vi "Libray.Connect_to_SNDB.vi"(0 "Log In Data":cluster{"Username":string, "Password":string}, 1 "Command":T2=enum."Initialize HTTPS", 2 "Curl":string="https://srv-sndb.iesy.com", 5 "Serial Number":string, 7 "Update step":T1, 11 "Fehler (Eingang, kein Fehler)":errorcluster, 12 "Input String":string, 13 "Type of the uploaded file":enum16{"txt", "pdf", "image/jpeg"}(ring)) -> (4 "Successful?":bool, 6 "body":string, 8 "headers":string, 15 "error out":errorcluster)   [LabVIEW 2026, in "Connect_to_SNDB_library.lvlib"]
uses:
  Connect_to_SNDB_library.lvlib
  Libray.Connect_to_SNDB_Command.ctl
  <vilib>/httpClient/ClientHandle.ctl
  <vilib>/JDP Science/JSONtext/Next JSON Value.vi
  <vilib>/JDP Science/JSONtext/String Subset.vi
  <vilib>/JDP Science/JSONtext/support/Strip Quotes and Unescape.vi
  <vilib>/JDP Science/JSONtext/Parsing/Advance past next JSON Value (inlined COPY).vi
  <vilib>/JDP Science/JSONtext/support/Unescape JSON string.vi
  <vilib>/JDP Science/JSONtext/Parsing/Advance past whitespace.vi
  <vilib>/JDP Science/JSONtext/Parsing/Advance past String.vi
  <vilib>/JDP Science/JSONtext/Parsing/Advance past Number.vi
  <vilib>/JDP Science/JSONtext/Parsing/Advance past Line Ending.vi
  <vilib>/JDP Science/JSONtext/support/Format JSON Object.vi
  <vilib>/httpClient/POSTBuffer.vi
  <vilib>/JDP Science/JSONtext/Parsing/Parse Full Path or Item Name.vi
  <vilib>/JDP Science/JSONtext/Parsing/Advance past Array.vi
  <vilib>/JDP Science/JSONtext/Parsing/Advance past Object.vi
  <vilib>/JDP Science/JSONtext/support/Error Cluster From Code.vi
  <vilib>/JDP Science/JSONtext/Offset/Find Item Locations by Path.vi
  <vilib>/httpClient/LabVIEWHTTPClient.lvlib
  <vilib>/JDP Science/JSONtext/JSONtext.lvlib
panel:
  out "MAC_Status_Array(with\"\")":string[](array[string])
  out "MAC_Array(with\"\")":string[](array[string])
  out "-H":string
  # "SNDB Libray"
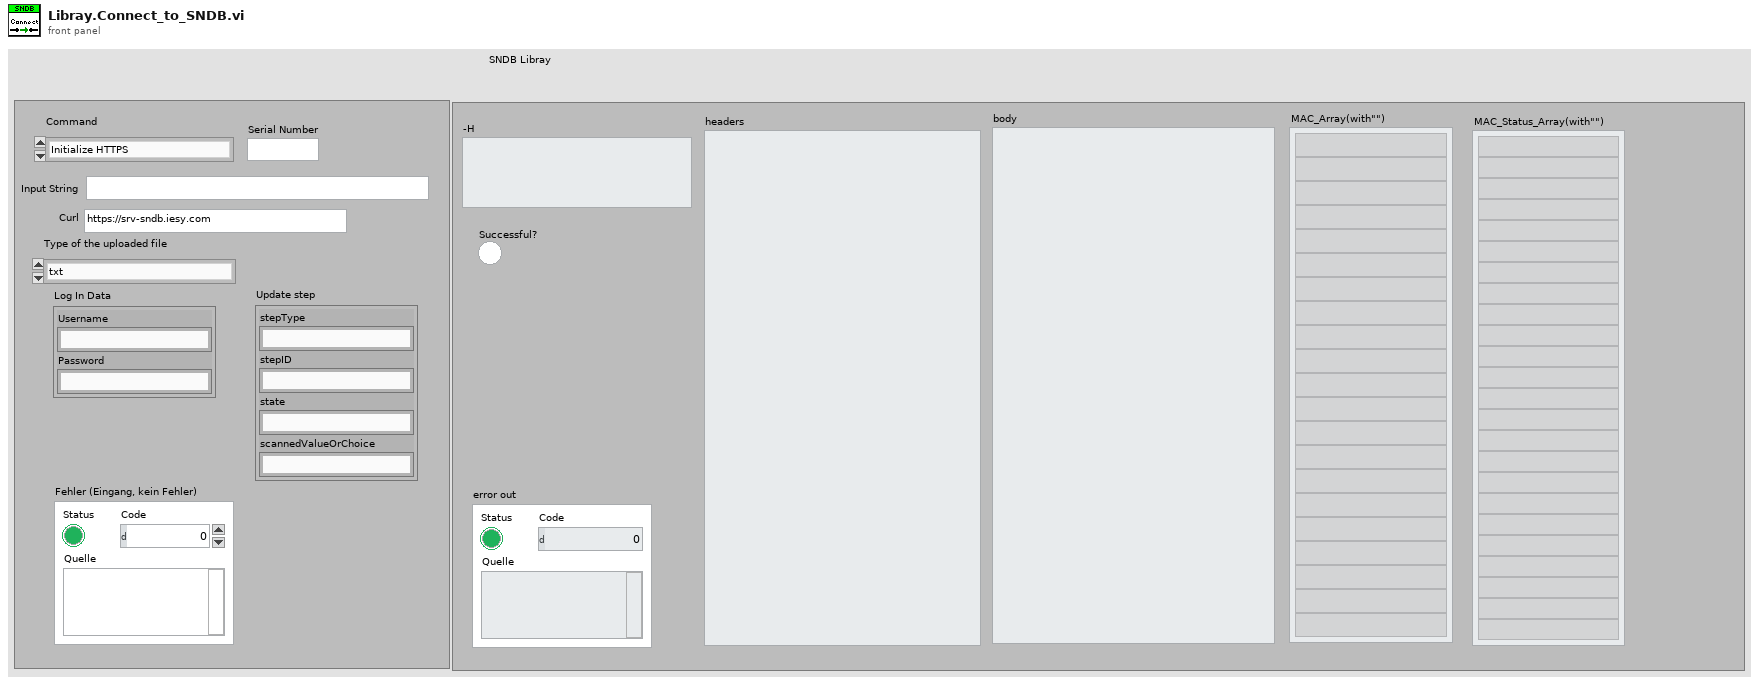
[diagram p1: front panel]
types:
  T1 = cluster{"stepType":string, "stepID":string, "state":string, "scannedValueOrChoice":string}
  T2 = typedef "Connect_to_SNDB_library.lvlib/Libray.Connect_to_SNDB_Command.ctl" = enum16{"No command", "Initialize HTTPS", "Authentication: Creat a token", "Authentication: Get all tokens", "Authentication: Revoke the token", "Label: Creat a label configuration", "Label: Get all configured labels", "Label: Update the label configuration", "Label: Delete the label configuration", "Label: Creat a colour ribbon", "Label: Update the colour ribbon", "Label: Get all colour ribbons", "Label: Delete the colour ribbon", "Label: Creat a label tape", "Label: Update the label tape", "Label: Get all label tapes", "Label: Delete the label tape", "Label: Get all label parameters", "Product: Get all product informations", "Product: Get all reading steps", "Seriennummer: Update the info text", "Seriennummer: Set all step states open", "Seriennummer: Update step states", "Seriennummer: Get data and steps", "Seriennummer: Get all label configurations", "Seriennummer: Create a text report(Prüfbericht)", "Seriennummer: Get the text report(Prüfbericht)", "Seriennummer: Delete the text report(Prüfbericht)", "Seriennummer: Upload a document(txt file)", "Seriennummer: Get the document", "Seriennummer: Get the document thumbnail", "Seriennummer: Delete the document", "Seriennummer: Bulk lookup", "Vorgang: Update the description text", "Vorgang: Migrate serial numbers to a Vorgang", "Vorgang: Migrate serial numbers to a product revision", "Vorgang: Update step states", "Vorgang: Create test reports(Prüfprotokoll)", "Vorgang: Get basic data", "Vorgang: Get serial number data and steps", "Vorgang: Get all serial numbers", "Vorgang: Generate a CSV file", "Vorgang: Generate an XLSX file", "Vorgang: Get a CSV file(Fertigmeldung report)", "Fertigmeldung: Create a Fertigmeldung", "Fertigmeldung: Revert the Fertigmeldung", "User: Get all users", "User: Update an user", "User: Get a single user", "User: Get all user roles", "User: Update a user role", "User: Get a single user role", "User: Get all permissions", "Search: Get Vorgang/Produkt combinations", "Search: Get Vorgang/Produkt/SN combinations", "Search: Get Seriennummern by Vorgang and Produkt", "Search: Lookup Vorgang", "MAC addresses: Get all reserved MAC addresses", "MAC addresses: Get the most recently reserved MAC addresses", "MAC addresses: Get data for a MAC address", "MAC addresses: Reserve a number of MAC addresses for a Seriennummer", "MAC addresses: Make a reserved MAC address as flashed", "Deinitialize HTTPs"}
  T3 = typedef "LabVIEWHTTPClient.lvlib/ClientHandle.ctl" = refnum<k1>
  T4 = cluster{"Name":string, "Value":string, "File":path, "Filename":string, "MIME type":string}
  T5 = cluster{"Name":string, "Value":string, "File":path, "Filename":string, "MIME type":string}[]
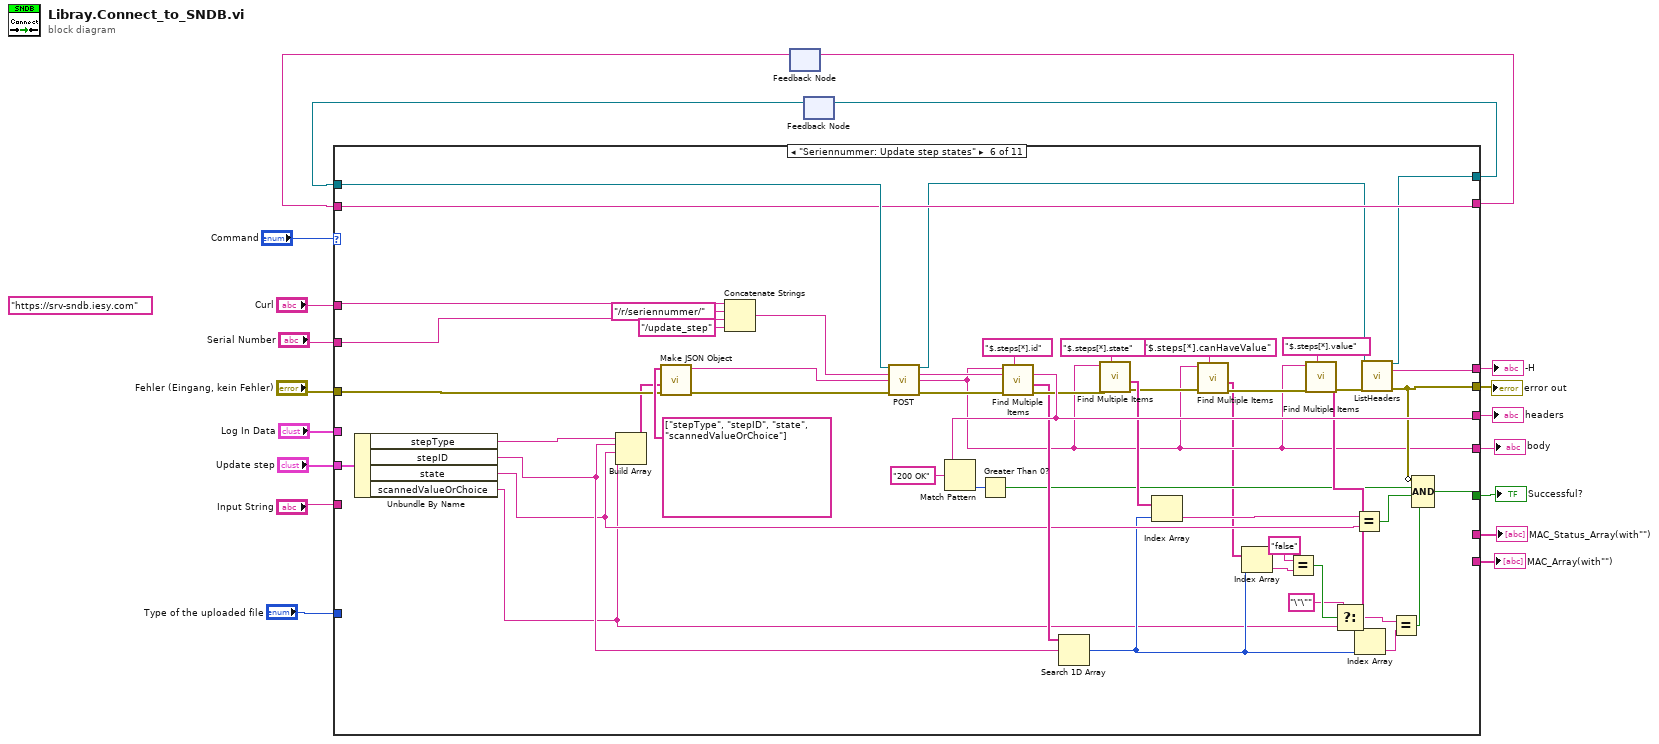
[diagram p0: block diagram]
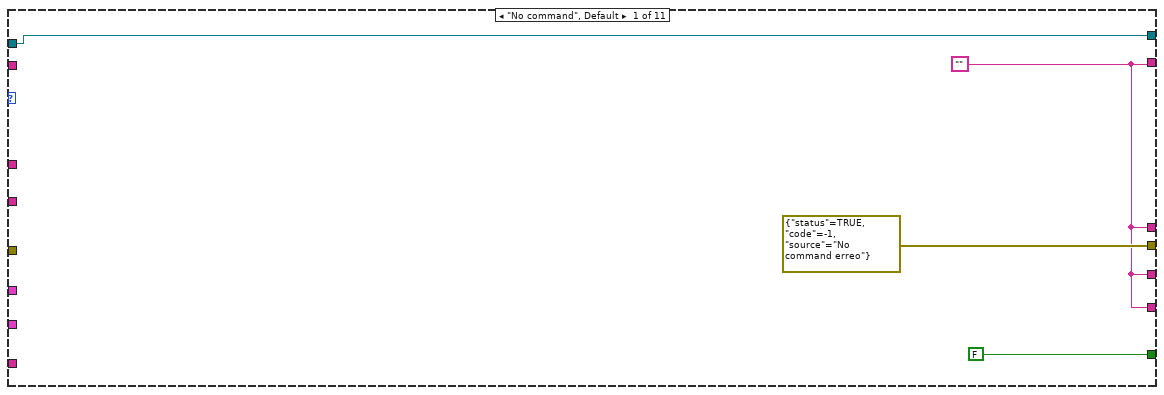
[diagram p2: hidden frame]
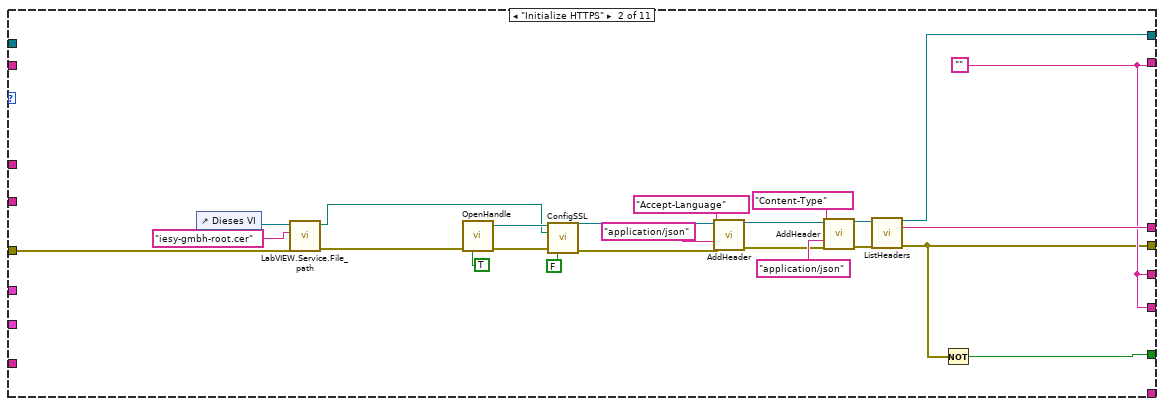
[diagram p3: hidden frame]
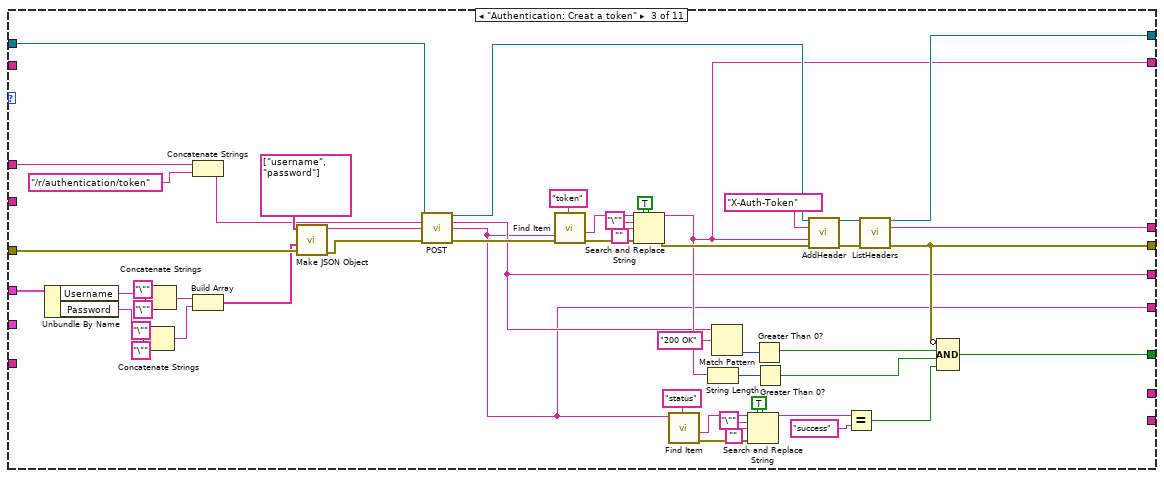
[diagram p4: hidden frame]
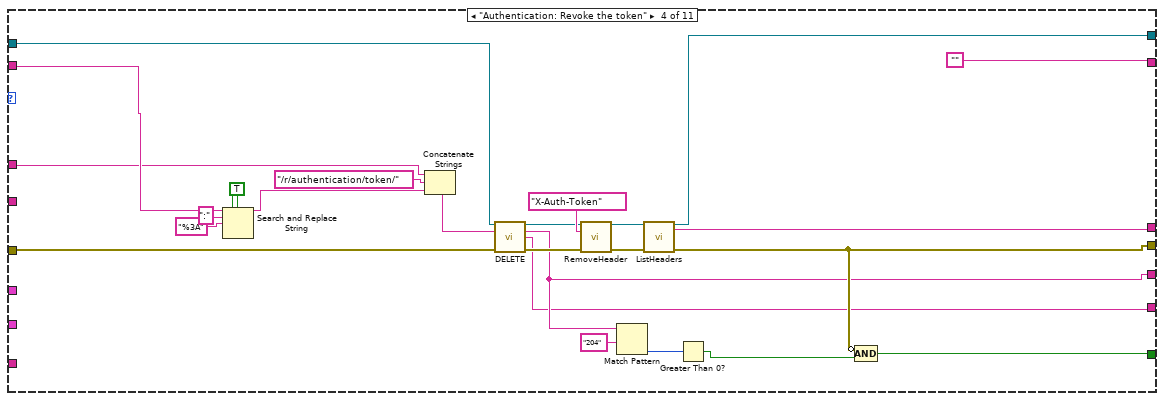
[diagram p5: hidden frame]
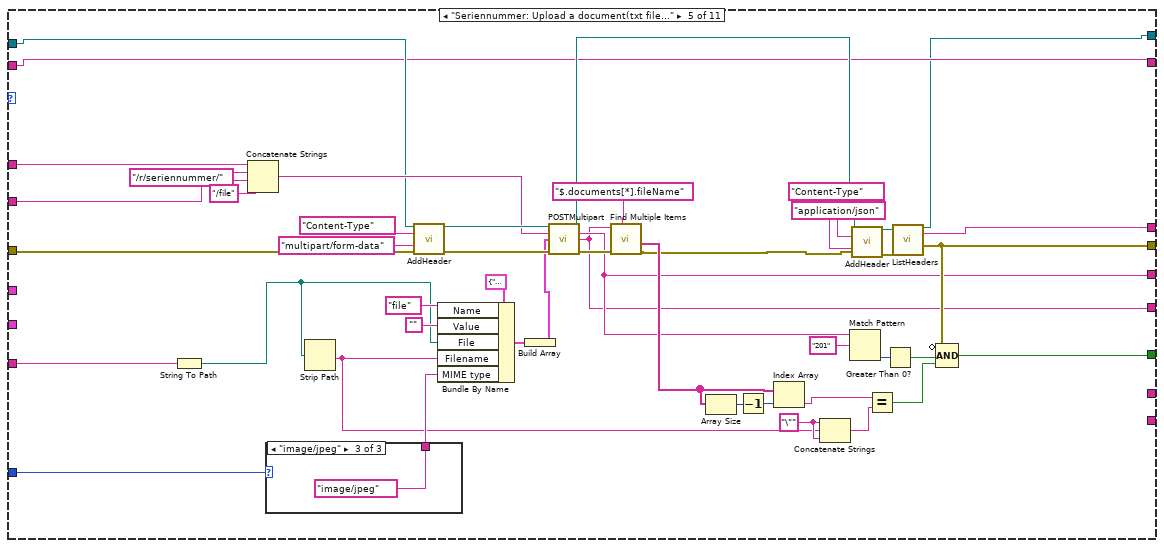
[diagram p6: hidden frame]
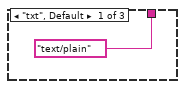
[diagram p7: hidden frame]
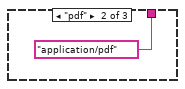
[diagram p8: hidden frame]
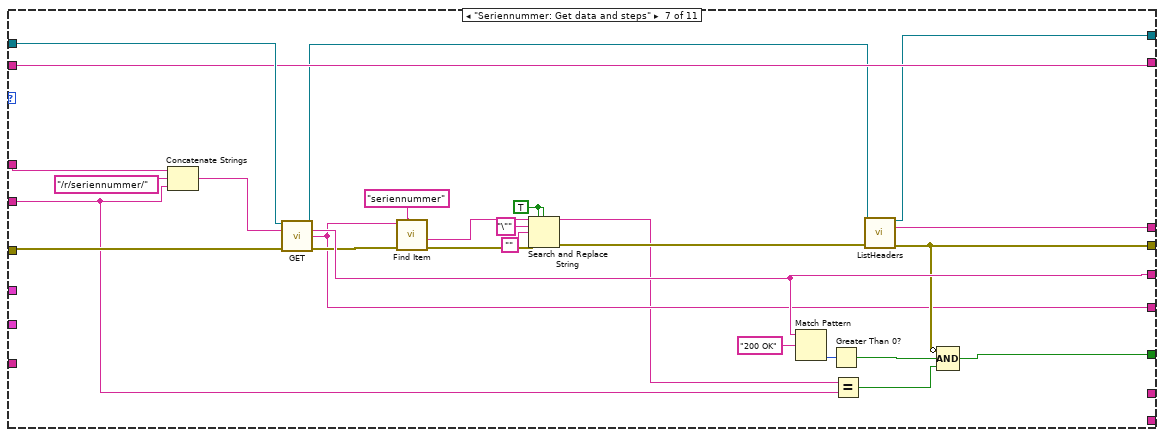
[diagram p9: hidden frame]
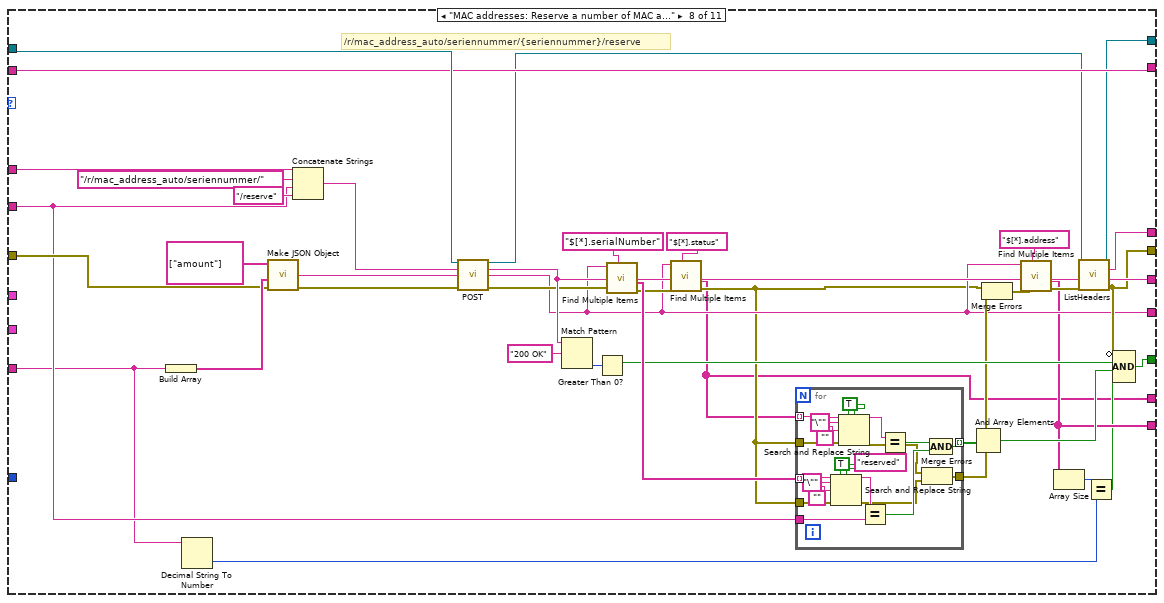
[diagram p10: hidden frame]
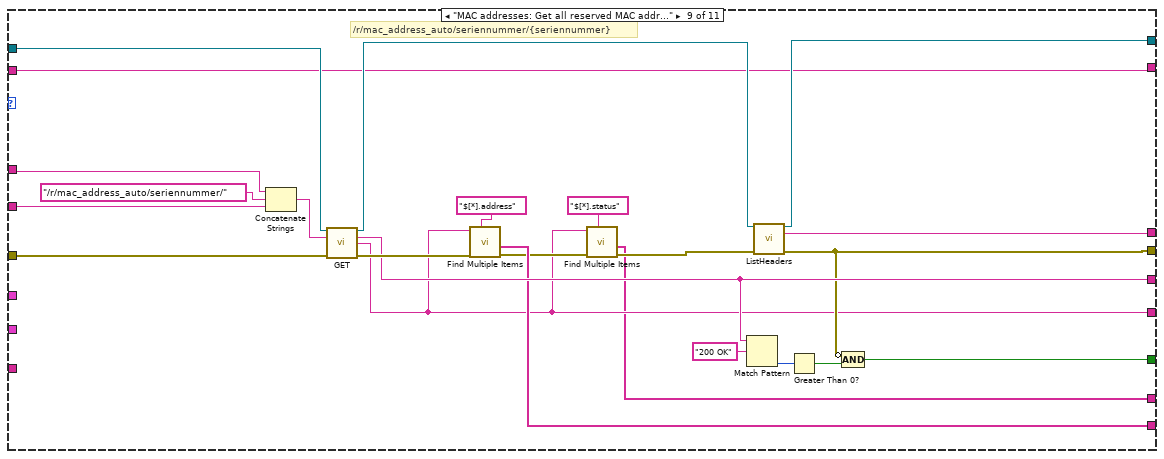
[diagram p11: hidden frame]
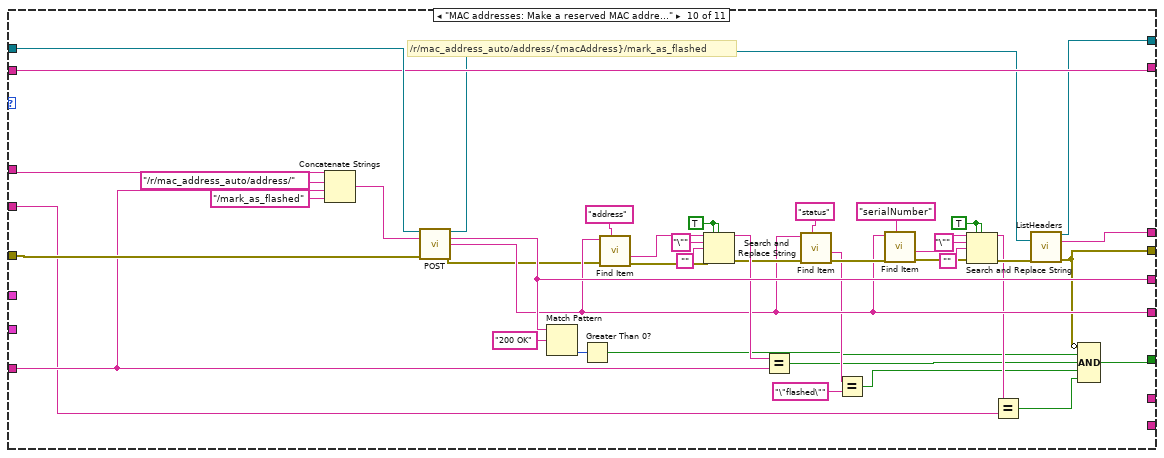
[diagram p12: hidden frame]
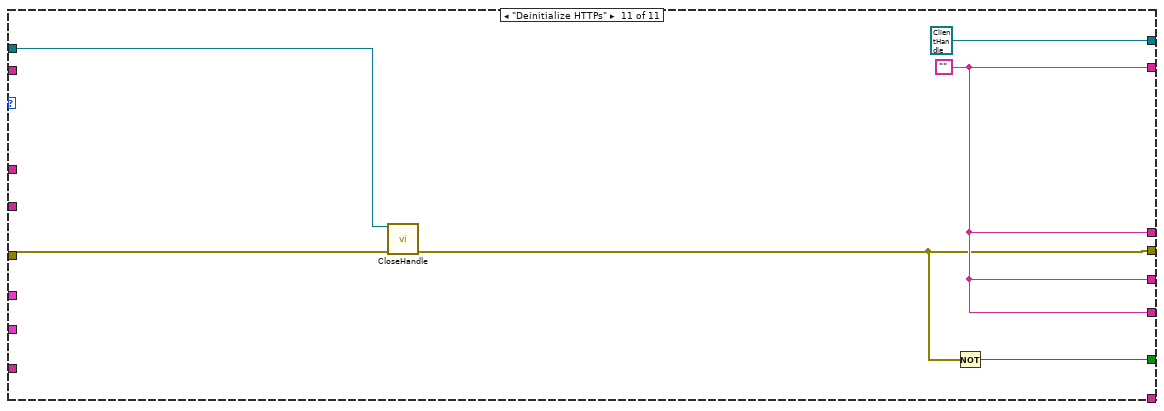
[diagram p13: hidden frame]
diagram:
  (unwired) "https://srv-sndb.iesy.com" ("String")
  n1 = feedback #1() -> (w11:string)  [unwired: 1 in]
  n2 = feedback #2() -> (w16:T3)  [unwired: 1 in]
  n3 = case shown="\"Seriennummer: Update step states\"" "Command" {
    tunnel: "Fehler (Eingang, kein Fehler)" -> [_ w29 w68 w107 w134 w217 w244 w278 w320 w370 w380]
    tunnel: [errorcluster {"status"=TRUE, "code"=-1, "source"="No command erreo"} ("error out") w25 w56 w106 w133 w192 w240 w260 w315 w340 w378] -> w7
    tunnel: [w23 w28 w69 w108 w137 w194 w235 w257 w324 w335 T3 refnum ("client handle out")] -> w17
    tunnel: w16 -> [w23 _ w70 w109 w139 w219 w247 w285 w325 w372 w382]
    tunnel: [w20 w27 w57 w104 w129 w195 w236 w274 w319 w334 w379] -> w15
    tunnel: "Log In Data" -> [_ _ w67 _ _ _ _ _ _ _ _]
    tunnel: [FALSE w24 w52 w105 w132 w188 w239 w259 w316 w336 w377] -> w13
    tunnel: [w20 w26 w51 "" w138 w218 w246 w284 w323 w371 w379] -> w12
    tunnel: w11 -> [_ _ _ w102 w138 w218 w246 w284 w323 w371 _]
    tunnel: "Curl" -> [_ _ w50 w101 w136 w211 w248 w287 w322 w374 _]
    tunnel: [w20 w26 w49 w100 w131 w209 w241 w276 w318 w367 w379] -> w10
    tunnel: [w20 w26 w48 w99 w130 w181 w228 w258 w311 w354 w379] -> w9
    tunnel: "Serial Number" -> [_ _ _ _ w135 w210 w224 w269 w321 w342 _]
    tunnel: "Input String" -> [_ _ _ _ w125 _ _ w254 _ w359 _]
    tunnel: "Type of the uploaded file" -> [_ _ _ _ w124 _ _ _ _ _ _]
    tunnel: "Update step" -> [_ _ _ _ _ w208 _ _ _ _ _]
    tunnel: [_ _ _ _ _ _ _ w255 w317 _ _] -> w2
    tunnel: [_ _ _ _ _ _ _ w250 w310 _ _] -> w1
    frame "No command", Default {
      w20 = ""
    }
    frame "Initialize HTTPS" {
      w26 = ""
      n4 = control-ref of="Dieses VI"() -> (w33:refnum<vi>)
      n5 = call "LabVIEW.Service.File_path.vi"("Fehler (Eingang, kein Fehler)"=w29, "File name"="iesy-gmbh-root.cer" ("String"), "VI Reference"=w33) -> ("Fehler (Ausgang)"=w30:errorcluster, "Dateipfad-Bedienelement"=w31:path)  [unwired: 7 in]
      n6 = call <vilib>:"OpenHandle.vi"("error in (no error)"=w30, "verify server(true)"=TRUE) -> ("client handle out"=w45:T3, "error out"=w43:errorcluster)  [unwired: 12 in]
      n7 = call <vilib>:"ConfigSSL.vi"("client handle"=w45, "CA certificate file"=w31, "error in (no error)"=w43, "verify server (true)"=FALSE) -> ("client handle out"=w46:T3, "error out"=w44:errorcluster)  [unwired: 10 in]
      n8 = call <vilib>:"AddHeader.vi"("client handle"=w46, "header"="Accept-Language", "value"="application/json", "error in (no error)"=w44) -> ("client handle out"=w39:T3, "error out"=w40:errorcluster)  [unwired: 10 in]
      n9 = call <vilib>:"AddHeader.vi"("client handle"=w39, "header"="Content-Type", "value"="application/json", "error in (no error)"=w40) -> ("client handle out"=w34:T3, "error out"=w35:errorcluster)  [unwired: 10 in]
      n10 = call <vilib>:"ListHeaders.vi"("client handle"=w34, "error in (no error)"=w35) -> ("client handle out"=w28:T3, "headers"=w27:string, "error out"=w25:errorcluster)  [unwired: 11 in]
      n11 = Not(x=w25) -> (.not. x?=w24:bool)
    }
    frame "Authentication: Creat a token" {
      w77 = TRUE ("Alle ersetzen? (F)")
      w94 = TRUE ("Alle ersetzen? (F)")
      n12 = Unbundle By Name(w67) -> ("Username"=w60:string, "Password"=w59:string)
      n13 = Concatenate Strings("\"" ("String"), w59, "\"" ("String")) -> (w62:string)
      n14 = Concatenate Strings("\"" ("String"), w60, "\"" ("String")) -> (w61:string)
      n15 = Concatenate Strings(w50, "/r/authentication/token" ("String")) -> (w72:string)
      n16 = Build Array(w61, w62) -> (w58:string[])
      n17 = call <vilib>:"Make JSON Object.vi"("error in (no error)"=w68, "JSON Items"=w58, "Item Names"=string[] ["username", "password"]) -> ("error out"=w97:errorcluster, "<JSON>"=w71:string)  [unwired: 7 in]
      n18 = call-poly <vilib>:"POST.vi"("client handle"=w70, "url"=w72, "buffer"=w71, "error in (no error)"=w97) -> ("client handle out"=w88:T3, "headers"=w49:string, "body"=w48:string, "error out"=w95:errorcluster)  [unwired: 8 in]
      n19 = call <vilib>:"Find Item.vi"("$Path or Item Name"="token", "error in (no error)"=w95, "JSON"=w48) -> ("error out"=w90:errorcluster, "<JSON>"=w91:string)  [unwired: 5 in, 2 out]
      n20 = Search and Replace String(replace all?=w94, case sensitive?=w94, input string=w91, search string="\"" ("Such-String"), replace string="", error in=w90) -> (result string=w51:string, error out=w87:errorcluster)  [unwired: 2 in, 2 out]
      n21 = call <vilib>:"Find Item.vi"("$Path or Item Name"="status", "JSON"=w48) -> ("error out"=w81:errorcluster, "<JSON>"=w80:string)  [unwired: 6 in, 2 out]
      n22 = String Length(string=w51) -> (length=w82:i32)
      n23 = Match Pattern(string=w49, regular expression="200 OK" ("Regulärer Ausdruck")) -> (offset past match=w83:i32)  [unwired: 1 in, 3 out]
      n24 = Search and Replace String(replace all?=w77, case sensitive?=w77, input string=w80, search string="\"" ("Such-String"), replace string="", error in=w81) -> (result string=w75:string)  [unwired: 2 in, 3 out]
      n25 = Greater Than 0?(x=w83) -> (x > 0?=w55:bool)
      n26 = Greater Than 0?(x=w82) -> (x > 0?=w54:bool)
      n27 = call <vilib>:"AddHeader.vi"("client handle"=w88, "header"="X-Auth-Token", "value"=w51, "error in (no error)"=w87) -> ("client handle out"=w86:T3, "error out"=w85:errorcluster)  [unwired: 10 in]
      n28 = Equal?(x=w75, y="success" ("$Path or Item Name")) -> (x = y?=w53:bool)
      n29 = call <vilib>:"ListHeaders.vi"("client handle"=w86, "error in (no error)"=w85) -> ("client handle out"=w69:T3, "headers"=w57:string, "error out"=w56:errorcluster)  [unwired: 11 in]
      n30 = Compound Arithmetic op=AND ("Mehrfacharithmetik")(invert w56, w55, w54, w53) -> (w52:bool)
    }
    frame "Authentication: Revoke the token" {
      w122 = TRUE ("Alle ersetzen? (F)")
      n31 = Search and Replace String(replace all?=w122, case sensitive?=w122, input string=w102, search string=":" ("Such-String"), replace string="%3A" ("Such-String")) -> (result string=w119:string)  [unwired: 3 in, 3 out]
      n32 = Concatenate Strings(w101, "/r/authentication/token/", w119) -> (w110:string)
      n33 = call <vilib>:"DELETE.vi"("client handle"=w109, "url"=w110, "error in (no error)"=w107) -> ("client handle out"=w111:T3, "headers"=w100:string, "body"=w99:string, "error out"=w114:errorcluster)  [unwired: 9 in]
      n34 = call <vilib>:"RemoveHeader.vi"("client handle"=w111, "header"="X-Auth-Token", "error in (no error)"=w114) -> ("client handle out"=w112:T3, "error out"=w113:errorcluster)  [unwired: 11 in]
      n35 = Match Pattern(string=w100, regular expression="204") -> (offset past match=w118:i32)  [unwired: 1 in, 3 out]
      n36 = call <vilib>:"ListHeaders.vi"("client handle"=w112, "error in (no error)"=w113) -> ("client handle out"=w108:T3, "headers"=w104:string, "error out"=w106:errorcluster)  [unwired: 11 in]
      n37 = Greater Than 0?(x=w118) -> (x > 0?=w116:bool)
      n38 = Compound Arithmetic op=AND ("Mehrfacharithmetik")(invert w106, w116) -> (w105:bool)
    }
    frame "Seriennummer: Upload a document(txt file)" {
      w154 = "\"" ("String")
      n39 = String To Path(string=w125) -> (path=w126:path)
      n40 = Concatenate Strings(w136, "/r/seriennummer/", w135, "/file" ("String")) -> (w141:string)
      n41 = case shown="\"image/jpeg\"" w124 {
        tunnel: ["text/plain" ("MIME type") "application/pdf" ("MIME type") "image/jpeg" ("MIME type")] -> w164
        frame "txt", Default {
        }
        frame "pdf" {
        }
        frame "image/jpeg" {
        }
      }
      n42 = Strip Path(path=w126) -> (name=w127:string)  [unwired: 1 out]
      n43 = call <vilib>:"AddHeader.vi"("client handle"=w139, "header"="Content-Type", "value"="multipart/form-data", "error in (no error)"=w134) -> ("client handle out"=w160:T3, "error out"=w159:errorcluster)  [unwired: 10 in]
      n44 = Bundle By Name(cluster=T4 {"Name"="serial", "Value"="04IA01267", "File"=path "", "Filename"="", "MIME type"="application/octet-stream"} ("Element"), "Name"="file", "Value"="", "File"=w126, "Filename"=w127, "MIME type"=w164) -> (w161:T4)
      n45 = Build Array(w161) -> (w140:T5)
      n46 = call <vilib>:"POSTMultipart.vi"("client handle"=w160, "url"=w141, "data"=w140, "error in (no error)"=w159) -> ("client handle out"=w147:T3, "headers"=w131:string, "body"=w130:string, "error out"=w155:errorcluster)  [unwired: 8 in]
      n47 = call <vilib>:"Find Multiple Items.vi"("$Path or Item Name"="$.documents[*].fileName", "error in (no error)"=w155, "JSON"=w130) -> ("error out"=w128:errorcluster, "<JSON>"=w143:string[])  [unwired: 5 in, 2 out]
      n48 = Array Size(array=w143) -> (size(s)=w145:i32)
      n49 = Decrement(x=w145) -> (x-1=w144:i32)
      n50 = Index Array(array=w143, index=w144) -> (element=w142:string)
      n51 = Concatenate Strings(w154, w127, w154) -> (w153:string)
      n52 = Match Pattern(string=w131, regular expression="201" ("Regulärer Ausdruck")) -> (offset past match=w157:i32)  [unwired: 1 in, 3 out]
      n53 = call <vilib>:"AddHeader.vi"("client handle"=w147, "header"="Content-Type", "value"="application/json", "error in (no error)"=w128) -> ("client handle out"=w146:T3, "error out"=w148:errorcluster)  [unwired: 10 in]
      n54 = Equal?(x=w142, y=w153) -> (x = y?=w151:bool)
      n55 = Greater Than 0?(x=w157) -> (x > 0?=w152:bool)
      n56 = call <vilib>:"ListHeaders.vi"("client handle"=w146, "error in (no error)"=w148) -> ("client handle out"=w137:T3, "headers"=w129:string, "error out"=w133:errorcluster)  [unwired: 11 in]
      n57 = Compound Arithmetic op=AND ("Mehrfacharithmetik")(invert w133, w152, w151) -> (w132:bool)
    }
    frame "Seriennummer: Update step states" {
      n58 = Unbundle By Name(w208) -> ("stepType"=w187:string, "stepID"=w186:string, "state"=w185:string, "scannedValueOrChoice"=w173:string)
      n59 = Build Array(w187, w186, w185, w173) -> (w207:string[])
      n60 = call <vilib>:"Make JSON Object.vi"("error in (no error)"=w217, "JSON Items"=w207, "Item Names"=string[] ["stepType", "stepID", "state", "scannedValueOrChoice"]) -> ("error out"=w214:errorcluster, "<JSON>"=w212:string)  [unwired: 7 in]
      n61 = Concatenate Strings(w211, "/r/seriennummer/" ("String"), w210, "/update_step" ("String")) -> (w213:string)
      n62 = call-poly <vilib>:"POST.vi"("client handle"=w219, "url"=w213, "buffer"=w212, "error in (no error)"=w214) -> ("client handle out"=w193:T3, "headers"=w209:string, "body"=w181:string, "error out"=w205:errorcluster)  [unwired: 8 in]
      n63 = Match Pattern(string=w209, regular expression="200 OK" ("Regulärer Ausdruck")) -> (offset past match=w220:i32)  [unwired: 1 in, 3 out]
      n64 = Greater Than 0?(x=w220) -> (x > 0?=w191:bool)
      n65 = call <vilib>:"Find Multiple Items.vi"("$Path or Item Name"="$.steps[*].id", "error in (no error)"=w205, "JSON"=w181) -> ("error out"=w203:errorcluster, "<JSON>"=w201:string[])  [unwired: 5 in, 2 out]
      n66 = Search 1D Array(1D array=w201, element=w186) -> (index of element=w179:i32)  [unwired: 1 in]
      n67 = call <vilib>:"Find Multiple Items.vi"("$Path or Item Name"="$.steps[*].state", "error in (no error)"=w203, "JSON"=w181) -> ("error out"=w183:errorcluster, "<JSON>"=w200:string[])  [unwired: 5 in, 2 out]
      n68 = Index Array(array=w200, index=w179) -> (element=w198:string)
      n69 = call <vilib>:"Find Multiple Items.vi"("$Path or Item Name"="$.steps[*].canHaveValue", "error in (no error)"=w183, "JSON"=w181) -> ("error out"=w182:errorcluster, "<JSON>"=w180:string[])  [unwired: 5 in, 2 out]
      n70 = Index Array(array=w180, index=w179) -> (element=w177:string)
      n71 = Equal?(x="false", y=w177) -> (x = y?=w176:bool)
      n72 = call <vilib>:"Find Multiple Items.vi"("$Path or Item Name"="$.steps[*].value", "error in (no error)"=w182, "JSON"=w181) -> ("error out"=w196:errorcluster, "<JSON>"=w199:string[])  [unwired: 5 in, 2 out]
      n73 = Select(t="\"\"", s=w176, f=w173) -> (s? t:f=w175:string)
      n74 = Equal?(x=w198, y=w185) -> (x = y?=w190:bool)
      n75 = Index Array(array=w199, index=w179) -> (element=w197:string)
      n76 = call <vilib>:"ListHeaders.vi"("client handle"=w193, "error in (no error)"=w196) -> ("client handle out"=w194:T3, "headers"=w195:string, "error out"=w192:errorcluster)  [unwired: 11 in]
      n77 = Equal?(x=w175, y=w197) -> (x = y?=w189:bool)
      n78 = Compound Arithmetic op=AND ("Mehrfacharithmetik")(invert w192, w191, w190, w189) -> (w188:bool)
    }
    frame "Seriennummer: Get data and steps" {
      w234 = TRUE ("Alle ersetzen? (F)")
      n79 = Concatenate Strings(w248, "/r/seriennummer/" ("String"), w224) -> (w245:string)
      n80 = call <vilib>:"GET.vi"("client handle"=w247, "url"=w245, "error in (no error)"=w244) -> ("client handle out"=w237:T3, "headers"=w241:string, "body"=w228:string, "error out"=w230:errorcluster)  [unwired: 9 in]
      n81 = call <vilib>:"Find Item.vi"("$Path or Item Name"="seriennummer", "error in (no error)"=w230, "JSON"=w228) -> ("error out"=w227:errorcluster, "<JSON>"=w229:string)  [unwired: 5 in, 2 out]
      n82 = Search and Replace String(replace all?=w234, case sensitive?=w234, input string=w229, search string="\"" ("Such-String"), replace string="", error in=w227) -> (result string=w225:string, error out=w226:errorcluster)  [unwired: 2 in, 2 out]
      n83 = Match Pattern(string=w241, regular expression="200 OK" ("Regulärer Ausdruck")) -> (offset past match=w242:i32)  [unwired: 1 in, 3 out]
      n84 = Greater Than 0?(x=w242) -> (x > 0?=w238:bool)
      n85 = Equal?(x=w225, y=w224) -> (x = y?=w223:bool)
      n86 = call <vilib>:"ListHeaders.vi"("client handle"=w237, "error in (no error)"=w226) -> ("client handle out"=w235:T3, "headers"=w236:string, "error out"=w240:errorcluster)  [unwired: 11 in]
      n87 = Compound Arithmetic op=AND ("Mehrfacharithmetik")(invert w240, w238, w223) -> (w239:bool)
    }
    frame "MAC addresses: Reserve a number of MAC addresses for a Seriennummer" {
      # "/r/mac_address_auto/seriennummer/{seriennummer}/reserve"
      n88 = Build Array(w254) -> (w282:string[])
      n89 = Decimal String To Number(string=w254) -> (number=w252:i32)  [unwired: 2 in, 1 out]
      n90 = call <vilib>:"Make JSON Object.vi"("error in (no error)"=w278, "JSON Items"=w282, "Item Names"=string[] ["amount"]) -> ("error out"=w277:errorcluster, "<JSON>"=w281:string)  [unwired: 7 in]
      n91 = Concatenate Strings(w287, "/r/mac_address_auto/seriennummer/" ("String"), w269, "/reserve" ("String")) -> (w286:string)
      n92 = call-poly <vilib>:"POST.vi"("client handle"=w285, "url"=w286, "buffer"=w281, "error in (no error)"=w277) -> ("client handle out"=w275:T3, "headers"=w276:string, "body"=w258:string, "error out"=w267:errorcluster)  [unwired: 8 in]
      n93 = Match Pattern(string=w276, regular expression="200 OK" ("Regulärer Ausdruck")) -> (offset past match=w279:i32)  [unwired: 1 in, 3 out]
      n94 = Greater Than 0?(x=w279) -> (x > 0?=w264:bool)
      n95 = call <vilib>:"Find Multiple Items.vi"("$Path or Item Name"="$[*].serialNumber", "error in (no error)"=w267, "JSON"=w258) -> ("error out"=w266:errorcluster, "<JSON>"=w270:string[])  [unwired: 5 in, 2 out]
      n96 = call <vilib>:"Find Multiple Items.vi"("$Path or Item Name"="$[*].status", "error in (no error)"=w266, "JSON"=w258) -> ("error out"=w256:errorcluster, "<JSON>"=w250:string[])  [unwired: 5 in, 2 out]
      n97 = for {
        tunnel: w270 -> [w306] mode=indexing
        tunnel: w269 -> [w304]
        tunnel: w250 -> [w300] mode=indexing
        tunnel: [w295] -> w268 mode=indexing
        tunnel: w256 -> [w294]
        tunnel: w256 -> [w293]
        tunnel: [w290] -> w263
        w303 = TRUE ("Alle ersetzen? (F)")
        w309 = TRUE ("Alle ersetzen? (F)")
        n98 = Search and Replace String(replace all?=w309, case sensitive?=w309, input string=w306, search string="\"" ("Such-String"), replace string="", error in=w293) -> (result string=w305:string, error out=w292:errorcluster)  [unwired: 2 in, 2 out]
        n99 = Search and Replace String(replace all?=w303, case sensitive?=w303, input string=w300, search string="\"" ("Such-String"), replace string="", error in=w294) -> (result string=w299:string, error out=w291:errorcluster)  [unwired: 2 in, 2 out]
        n100 = Equal?(x=w305, y=w304) -> (x = y?=w296:bool)
        n101 = Equal?(x=w299, y="reserved") -> (x = y?=w297:bool)
        n102 = Merge Errors(w291, w292) -> (w290:errorcluster)
        n103 = Compound Arithmetic op=AND ("Mehrfacharithmetik")(w297, w296) -> (w295:bool)
      }
      n104 = And Array Elements(Boolean array=w268) -> (logical AND=w265:bool)
      n105 = Merge Errors(w256, w263) -> (w262:errorcluster)
      n106 = call <vilib>:"Find Multiple Items.vi"("$Path or Item Name"="$[*].address", "error in (no error)"=w262, "JSON"=w258) -> ("error out"=w261:errorcluster, "<JSON>"=w255:string[])  [unwired: 5 in, 2 out]
      n107 = Array Size(array=w255) -> (size(s)=w253:i32)
      n108 = call <vilib>:"ListHeaders.vi"("client handle"=w275, "error in (no error)"=w261) -> ("client handle out"=w257:T3, "headers"=w274:string, "error out"=w260:errorcluster)  [unwired: 11 in]
      n109 = Equal?(x=w253, y=w252) -> (x = y?=w251:bool)
      n110 = Compound Arithmetic op=AND ("Mehrfacharithmetik")(invert w260, w264, w265, w251) -> (w259:bool)
    }
    frame "MAC addresses: Get all reserved MAC addresses" {
      # "/r/mac_address_auto/seriennummer/{seriennummer}"
      n111 = Concatenate Strings(w322, "/r/mac_address_auto/seriennummer/" ("String"), w321) -> (w326:string)
      n112 = call <vilib>:"GET.vi"("client handle"=w325, "url"=w326, "error in (no error)"=w320) -> ("client handle out"=w332:T3, "headers"=w318:string, "body"=w311:string, "error out"=w327:errorcluster)  [unwired: 9 in]
      n113 = call <vilib>:"Find Multiple Items.vi"("$Path or Item Name"="$[*].address", "error in (no error)"=w327, "JSON"=w311) -> ("error out"=w313:errorcluster, "<JSON>"=w317:string[])  [unwired: 5 in, 2 out]
      n114 = call <vilib>:"Find Multiple Items.vi"("$Path or Item Name"="$[*].status", "error in (no error)"=w313, "JSON"=w311) -> ("error out"=w312:errorcluster, "<JSON>"=w310:string[])  [unwired: 5 in, 2 out]
      n115 = Match Pattern(string=w318, regular expression="200 OK" ("Regulärer Ausdruck")) -> (offset past match=w330:i32)  [unwired: 1 in, 3 out]
      n116 = call <vilib>:"ListHeaders.vi"("client handle"=w332, "error in (no error)"=w312) -> ("client handle out"=w324:T3, "headers"=w319:string, "error out"=w315:errorcluster)  [unwired: 11 in]
      n117 = Greater Than 0?(x=w330) -> (x > 0?=w329:bool)
      n118 = Compound Arithmetic op=AND ("Mehrfacharithmetik")(invert w315, w329) -> (w316:bool)
    }
    frame "MAC addresses: Make a reserved MAC address as flashed" {
      w347 = TRUE ("Alle ersetzen? (F)")
      w366 = TRUE ("Alle ersetzen? (F)")
      # "/r/mac_address_auto/address/{macAddress}/mark_as_flashed"
      n119 = Concatenate Strings(w374, "/r/mac_address_auto/address/" ("String"), w359, "/mark_as_flashed" ("String")) -> (w373:string)
      n120 = call-poly <vilib>:"POST.vi"("client handle"=w372, "url"=w373, "error in (no error)"=w370) -> ("client handle out"=w353:T3, "headers"=w367:string, "body"=w354:string, "error out"=w352:errorcluster)  [unwired: 9 in]
      n121 = Match Pattern(string=w367, regular expression="200 OK" ("Regulärer Ausdruck")) -> (offset past match=w368:i32)  [unwired: 1 in, 3 out]
      n122 = Greater Than 0?(x=w368) -> (x > 0?=w341:bool)
      n123 = call <vilib>:"Find Item.vi"("$Path or Item Name"="address", "error in (no error)"=w352, "JSON"=w354) -> ("error out"=w361:errorcluster, "<JSON>"=w362:string)  [unwired: 5 in, 2 out]
      n124 = Search and Replace String(replace all?=w366, case sensitive?=w366, input string=w362, search string="\"" ("Such-String"), replace string="", error in=w361) -> (result string=w360:string, error out=w357:errorcluster)  [unwired: 2 in, 2 out]
      n125 = Equal?(x=w360, y=w359) -> (x = y?=w339:bool)
      n126 = call <vilib>:"Find Item.vi"("$Path or Item Name"="status", "error in (no error)"=w357, "JSON"=w354) -> ("error out"=w355:errorcluster, "<JSON>"=w351:string)  [unwired: 5 in, 2 out]
      n127 = Equal?(x=w351, y="\"flashed\"") -> (x = y?=w338:bool)
      n128 = call <vilib>:"Find Item.vi"("$Path or Item Name"="serialNumber", "error in (no error)"=w355, "JSON"=w354) -> ("error out"=w346:errorcluster, "<JSON>"=w344:string)  [unwired: 5 in, 2 out]
      n129 = Search and Replace String(replace all?=w347, case sensitive?=w347, input string=w344, search string="\"" ("Such-String"), replace string="", error in=w346) -> (result string=w343:string, error out=w345:errorcluster)  [unwired: 2 in, 2 out]
      n130 = Equal?(x=w343, y=w342) -> (x = y?=w337:bool)
      n131 = call <vilib>:"ListHeaders.vi"("client handle"=w353, "error in (no error)"=w345) -> ("client handle out"=w335:T3, "headers"=w334:string, "error out"=w340:errorcluster)  [unwired: 11 in]
      n132 = Compound Arithmetic op=AND ("Mehrfacharithmetik")(invert w340, w341, w339, w338, w337) -> (w336:bool)
    }
    frame "Deinitialize HTTPs" {
      w379 = ""
      n133 = call <vilib>:"CloseHandle.vi"("client handle"=w382, "error in (no error)"=w380) -> ("error out"=w378:errorcluster)  [unwired: 13 in]
      n134 = Not(x=w378) -> (.not. x?=w377:bool)
    }
  }
  "-H" <- w15
  "Successful?" <- w13
  "headers" <- w10
  "body" <- w9
  "error out" <- w7
  "MAC_Array(with\"\")" <- w2
  "MAC_Status_Array(with\"\")" <- w1
  n135 = feedback-in #1(w12) -> ()
  n136 = feedback-in #2(w17) -> ()
